vi "TCP Check Connection.vi"(8 "error in (no error)":errorcluster, 11 "Connection In":T1) -> (0 "error out":errorcluster, 2 "Disconnected":bool, 3 "Connection out":T1)   [LabVIEW 2010]
doc: "This VI removes the host connection from the connection manager list if it becomes disconnected for any reason."
uses:
  stm_TCP Connection Info.ctl
  stm_MetaDataElement.ctl
  NI STM.lvlib
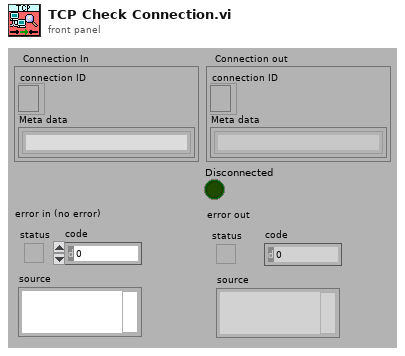
[diagram p1: front panel]
types:
  T1 = typedef "stm_TCP Connection Info.ctl" = cluster{"connection ID":refnum<k5>, "Meta data":T2[]}
  T2 = typedef "stm_MetaDataElement.ctl" = string
  T3 = typedef "NI STM.lvlib/TCP Connection Info.ctl" = cluster{"connection ID":refnum<k5>, "Meta data":T4[]}
  T4 = typedef "NI STM.lvlib/MetaDataElement.ctl" = string
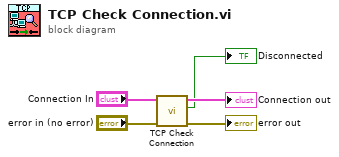
[diagram p0: block diagram]
diagram:
  n1 = call "TCP Check Connection.vi"("error in"="error in (no error)", "Connection In"="Connection In") -> ("error out"=→"error out":errorcluster, "Disconnected"=→"Disconnected":bool, "Connection out"=→"Connection out":T3)  [unwired: 7 in]
